vi "Prepare Project.vi"(8 "error in":errorcluster, 11 "G-CLI Runner in":refnum<class "Runner.lvclass">) -> (0 "error out":errorcluster, 3 "G-CLI Runner out":refnum<class "Runner.lvclass">)   [LabVIEW 2026, in "Runner.lvlib" / "Runner.lvclass"]
doc: "Prepare project based on project template."
uses:
  Runner.lvclass
  Runner.lvclass/Runner.ctl
  Interfaces/ILogger/ILogger Messages/Log Msg/Log Msg.lvclass/Log Msg.ctl
  <vilib>/ActorFramework/Message Enqueuer/Message Enqueuer.lvclass/Message Enqueuer.ctl
  <vilib>/ActorFramework/Message Enqueuer/Enqueue.vi
  Interfaces/ILogger/ILogger Messages/Log Msg/Log Msg.lvclass
  <vilib>/ActorFramework/Message Priority Queue/Priority Enqueue.vi
  Interfaces/IFile Manager/IFile Manager.lvclass
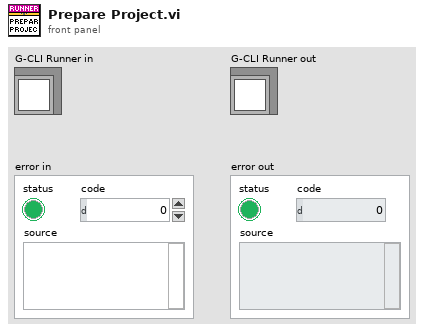
[diagram p1: front panel]
types:
  T1 = typedef "Log Entry--cluster.ctl" = cluster{"Time":timestamp, "Message":string}
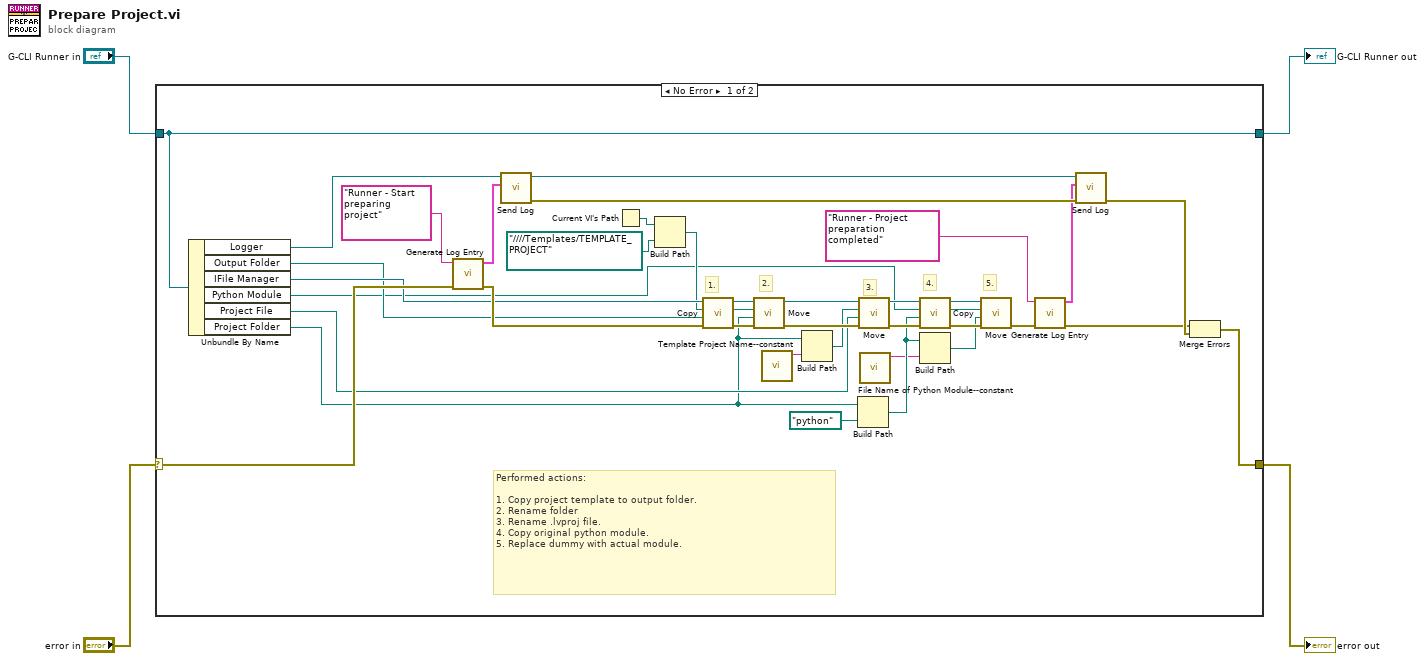
[diagram p0: block diagram]
diagram:
  n1 = case shown="No Error" "error in" {
    selector: "error in" -> [w32 w44]
    tunnel: [w42 w44] -> w4
    tunnel: "G-CLI Runner in" -> [w31 w43]
    tunnel: [w31 w43] -> w1
    frame No Error {
      # "Performed actions:\n\n1. Copy project template to output folder.\n2. Rename folder\n3. Rename .lvproj file.\n4. Copy original python module.\n5. Replace dummy with actual module."
      # "5."
      # "4."
      # "3."
      # "2."
      # "1."
      n2 = Unbundle By Name(w31) -> ("Logger"=w17:refnum<class "Message Enqueuer.lvclass">, "Output Folder"=w20:path, "IFile Manager"=w28:refnum<class "IFile Manager.lvclass">, "Python Module"=w19:path, "Project File"=w6:path, "Project Folder"=w5:path)
      n3 = call "Generate Log Entry.vi"("error in"=w32, "Message"="Runner - Start preparing project") -> ("error out"=w37:errorcluster, "Log Entry"=w15:T1)  [unwired: 8 in]
      n4 = call "Send Log.vi"("Log Entry"=w15, "Message Enqueuer"=w17) -> ("error out"=w36:errorcluster, "Message Enqueuer out"=w12:refnum<class "Message Enqueuer.lvclass">)  [unwired: 8 in]
      n5 = Current VI's Path() -> (path=w29:path)
      n6 = Build Path(base path=w29, name or relative path=path "../../../../Templates/TEMPLATE_PROJECT") -> (appended path=w27:path)
      n7 = call-dynamic "Copy.vi"("error in"=w37, "Target Folder"=w20, "Source File"=w27, "IFile Manager in"=w28) -> ("error out"=w40:errorcluster, "New Path"=w25:path, "IFile Manager out"=w26:refnum<class "IFile Manager.lvclass">)  [unwired: 5 in]
      n8 = call-dynamic "Move.vi"("error in"=w40, "Target"=w5, "Source"=w25, "IFile Manager in"=w26) -> ("error out"=w39:errorcluster, "IFile Manager out"=w24:refnum<class "IFile Manager.lvclass">)  [unwired: 6 in]
      n9 = call "Template Project Name--constant.vi"() -> ("Template Project Name"=w23:string)  [unwired: 11 in]
      n10 = Build Path(base path=w5, name or relative path=w23) -> (appended path=w22:path)
      n11 = Build Path(base path=w5, name or relative path=path "python") -> (appended path=w9:path)
      n12 = call-dynamic "Move.vi"("error in"=w39, "Target"=w6, "Source"=w22, "IFile Manager in"=w24) -> ("error out"=w38:errorcluster, "IFile Manager out"=w21:refnum<class "IFile Manager.lvclass">)  [unwired: 6 in]
      n13 = call "File Name of Python Module--constant.vi"() -> ("File Name of Python Module"=w7:string)  [unwired: 11 in]
      n14 = call-dynamic "Copy.vi"("error in"=w38, "Target Folder"=w9, "Source File"=w19, "IFile Manager in"=w21) -> ("error out"=w34:errorcluster, "New Path"=w10:path, "IFile Manager out"=w11:refnum<class "IFile Manager.lvclass">)  [unwired: 5 in]
      n15 = Build Path(base path=w9, name or relative path=w7) -> (appended path=w8:path)
      n16 = call-dynamic "Move.vi"("error in"=w34, "Target"=w8, "Source"=w10, "IFile Manager in"=w11) -> ("error out"=w33:errorcluster)  [unwired: 6 in, 1 out]
      n17 = call "Generate Log Entry.vi"("error in"=w33, "Message"="Runner - Project preparation completed") -> ("error out"=w35:errorcluster, "Log Entry"=w13:T1)  [unwired: 8 in]
      n18 = call "Send Log.vi"("error in (no error)"=w36, "Log Entry"=w13, "Message Enqueuer"=w12) -> ("error out"=w41:errorcluster)  [unwired: 7 in, 1 out]
      n19 = Merge Errors(w35, w41) -> (w42:errorcluster)
    }
    frame Error {
      # "Pass error without further actions."
    }
  }
  "error out" <- w4
  "G-CLI Runner out" <- w1
